vi "lab3_1_rt.vi"() -> ()   [LabVIEW 2025]
uses:
  <vilib>/rvi/interface/nirviMethod/nirviMethod.xnode
  <vilib>/rvi/errors/niLvFpgaMergeErrorWithErrorCode.vi
  <vilib>/rvi/interface/nirviCloseFPGA/nirviCloseFPGA.xnode
  <vilib>/FPGAPlugInAG/Dynamic/niLvFpga_ReadFifo_Dynamic.vi
  <vilib>/FPGAPlugInAG/Dynamic/niLvFpga_Close_Dynamic.vi
  <vilib>/dex/Flush And Wait Empty Condition.ctl
  vi/thresholds.ctl
panel:
  in  "Threshold":T1
  out "Elements Remaining":u32
  out "Waveform Graph":i16[][](graph)
  out "error out":errorcluster
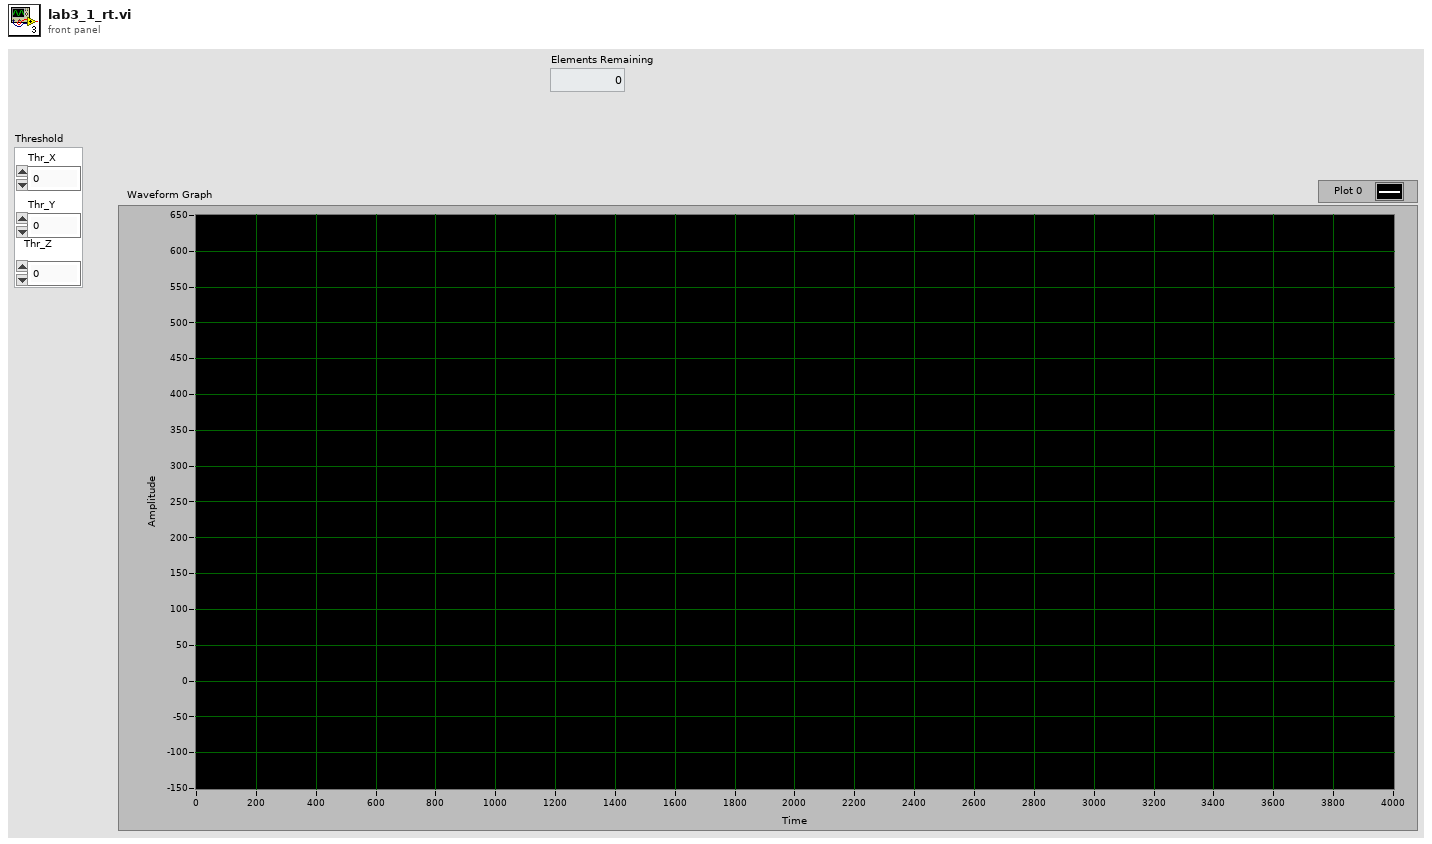
[diagram p1: front panel]
types:
  T1 = typedef "thresholds.ctl" = cluster{"Thr_X":i16, "Thr_Y":i16, "Thr_Z":i16}
  T2 = typedef "Flush And Wait Empty Condition.ctl" = u8
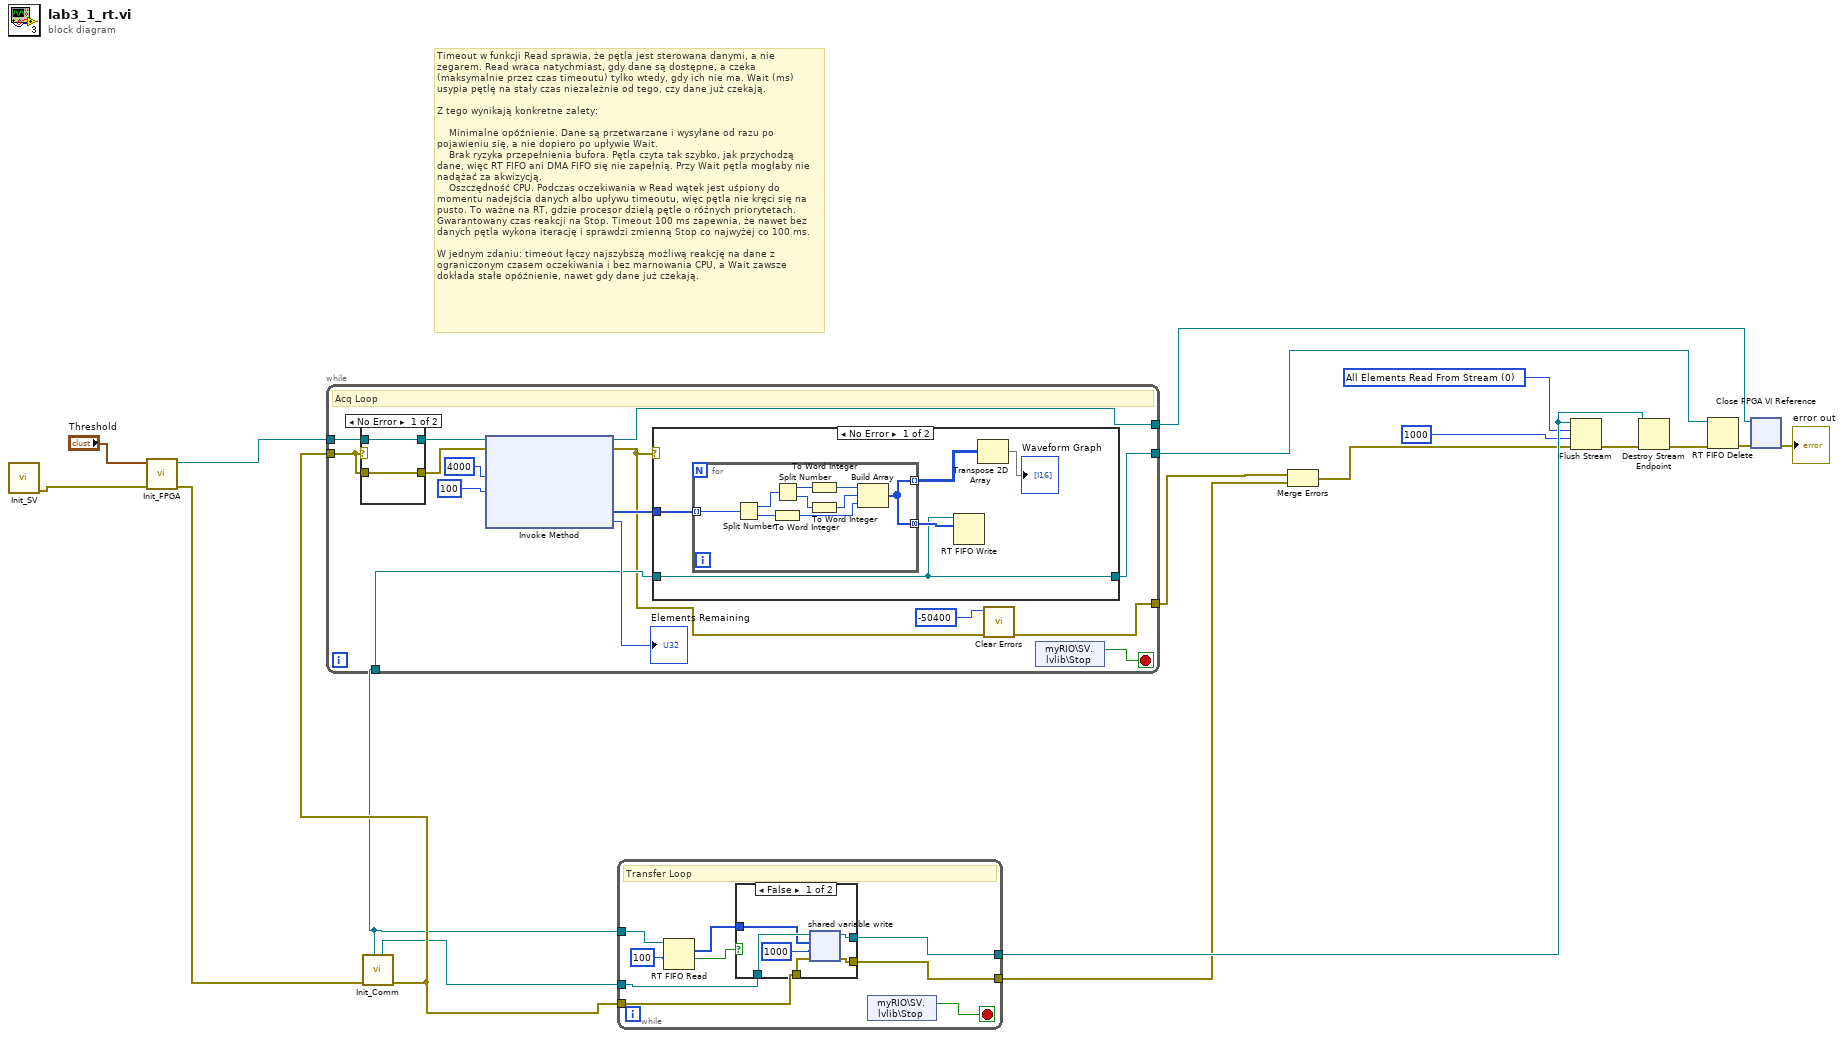
[diagram p0: block diagram]
diagram:
  w16 = T2 0 items=["All Elements Read From Stream", "All Elements Available for Reading"] ("wait condition")
  # "Timeout w funkcji Read sprawia, że pętla jest sterowana danymi, a nie zegarem. Read wraca natychmiast, gdy dane są dostępne, a czeka (maksymalnie przez czas timeoutu) tylko wtedy, gdy ich nie ma. Wait (ms) usypia pętlę na stały czas niezależnie od tego, czy dane już czekają.\n\nZ tego wynikają konkretne zalety:\n\n    Minimalne opóźnienie. Dane są przetwarzane i wysyłane od razu po pojawieniu się, a nie dopiero po upływie Wait.\n    Brak ryzyka przepełnienia bufora. Pętla czyta tak szybko, jak przychodzą dane, więc RT FIFO ani DMA FIFO się nie zapełnią. Przy Wait pętla mogłaby nie nadążać za akwizycją.\n    Oszczędność CPU. Podczas oczekiwania w Read wątek jest uśpiony do momentu nadejścia danych albo upływu timeoutu, więc pętla nie kręci się na pusto. To ważne na RT, gdzie procesor dzielą pętle o różnych priorytetach.\nGwarantowany czas reakcji na Stop. Timeout 100 ms zapewnia, że nawet bez danych pętla wykona iterację i sprawdzi zmienną Stop co najwyżej co 100 ms.\n\nW jednym zdaniu: timeout łączy najszybszą możliwą reakcję na dane z ograniczonym czasem oczekiwania i bez marnowania CPU, a Wait zawsze dokłada stałe opóźnienie, nawet gdy dane już czekają."
  n1 = call "Init_SV.vi"() -> ("error out"=w13:errorcluster)  [unwired: 11 in]
  n2 = call "Init_FPGA.vi"("error in"=w13, "Threshold"="Threshold") -> ("error out"=w10:errorcluster, "FPGA VI Reference Out"=w11:refnum<k20>)  [unwired: 8 in]
  n3 = call "Init_Comm.vi"("error in"=w10) -> ("error out"=w9:errorcluster, "writer endpoint ref out"=w8:refnum<k21>, "rt fifo ref out"=w3:refnum<k33>)  [unwired: 8 in]
  n4 = while {
    tunnel: w11 -> [w30]
    tunnel: w9 -> [w29]
    tunnel: [w28] -> w2
    tunnel: [w22] -> w6
    tunnel: w3 -> [w25]
    tunnel: [w20] -> w1
    stop <- w24 stop-if-true
    # "Acq Loop"
    n5 = case shown="No Error" w29 {
      tunnel: w30 -> [w51 w53]
      tunnel: [w51 w53] -> w34
      tunnel: w29 -> [w50 w52]
      tunnel: [w50 w52] -> w33
      frame No Error {
      }
      frame Error {
      }
    }
    n6 = xnode "Invoke Method"("FPGA VI Reference In"=w34, "error in"=w33, "Number of Elements"=u32 4000, "Timeout (ms)"=100) -> ("FPGA VI Reference Out"=w28:refnum<k20>, "error out"=w23:errorcluster, "Data"=w27:u64[], "Elements Remaining"=→"Elements Remaining":u32)
    n7 = case shown="No Error" w23 {
      tunnel: w27 -> [w39 _]
      tunnel: w25 -> [w35 w49]
      tunnel: [w35 w49] -> w20
      frame No Error {
        n8 = for {
          tunnel: w39 -> [w48] mode=indexing
          tunnel: [w40] -> w37 mode=concatenating
          tunnel: [w40] -> w36 mode=indexing
          n9 = Split Number(x=w48) -> (hi(x)=w47:u32, lo(x)=w44:u32)
          n10 = To Word Integer(number=w44) -> (16bit integer=w41:i16)
          n11 = Split Number(x=w47) -> (hi(x)=w46:u16, lo(x)=w45:u16)
          n12 = To Word Integer(number=w46) -> (16bit integer=w43:i16)
          n13 = To Word Integer(number=w45) -> (16bit integer=w42:i16)
          n14 = Build Array(w43, w42, w41) -> (w40:i16[])
        }
        n15 = RT FIFO Write(0:w35, 1:w37) -> ()  [unwired: 3 in, 4 out]
        n16 = Transpose 2D Array(2D array=w36) -> (transposed array=→"Waveform Graph":i16[][])
      }
      frame Error {
      }
    }
    n17 = call <vilib>:"Clear Errors.vi"("error in (no error)"=w23, "specific error code to clear (0: all)"=-50400) -> ("error out"=w22:errorcluster)  [unwired: 4 in, 1 out]
    n18 = shared-variable "myRIO\\SV.lvlib\\Stop"() -> (w24:bool)  [unwired: 1 in, 1 out]
  }
  n19 = while {
    tunnel: w3 -> [w62]
    tunnel: w8 -> [w59]
    tunnel: [w57] -> w18
    tunnel: [w56] -> w7
    tunnel: w9 -> [w58]
    stop <- w54 stop-if-true
    # "Transfer Loop"
    n20 = RT FIFO Read(0:w62, 2:100 ("timeout in ms (0)")) -> (9:w55:i16[], 10:w60:bool)  [unwired: 2 in, 3 out]
    n21 = case shown="False" w60 {
      tunnel: w59 -> [w68 w69]
      tunnel: w58 -> [w67 w70]
      tunnel: [w66 w69] -> w57
      tunnel: [w65 w70] -> w56
      tunnel: w55 -> [w63 _]
      frame False {
        n22 = shared-variable-write(w68, w67, w63, 1000 ("timeout ms (-1)")) -> (w66:refnum<k21>, w65:errorcluster)  [unwired: 1 out]
      }
      frame True {
      }
    }
    n23 = shared-variable "myRIO\\SV.lvlib\\Stop"() -> (w54:bool)  [unwired: 1 in, 1 out]
  }
  n24 = Merge Errors(w6, w7) -> (w5:errorcluster)
  n25 = Flush Stream(8:w5, 9:1000 ("timeout in ms (-1)"), 10:w16, 11:w18) -> (0:w17:errorcluster)  [unwired: 2 out]
  n26 = Destroy Stream Endpoint(8:w17, 11:w18) -> (0:w15:errorcluster)
  n27 = RT FIFO Delete(0:w1, 3:w15) -> (11:w14:errorcluster)  [unwired: 1 in]
  n28 = xnode "Close FPGA VI Reference"("FPGA VI Reference In"=w2, "error in"=w14) -> ("error out"=→"error out":errorcluster)
